vi "log queue utility.vi"(10 "array":string[](array[string]), 11 "queue with message cluster":refnum<queue>) -> (3 "appended array":string[](array[string]))   [LabVIEW 2025]
uses:
  support/Message Queue/Message Cluster_TICO behavior.ctl
panel:
  # "feed output array back into input array wiring node to create feedback element"
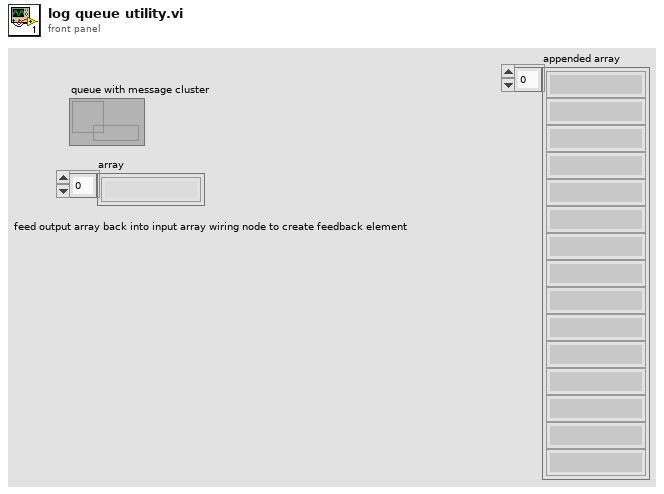
[diagram p1: front panel]
types:
  T1 = typedef "Message Cluster_TICO behavior.ctl" = cluster{"Message":string, "Message Data":variant}
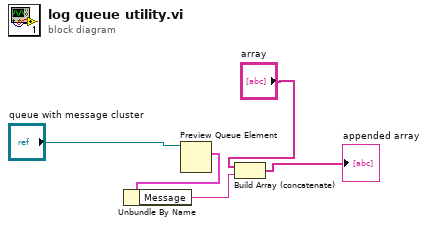
[diagram p0: block diagram]
diagram:
  n1 = Preview Queue Element(queue="queue with message cluster") -> (element=w3:T1)  [unwired: 2 in, 3 out]
  n2 = Unbundle By Name(w3) -> ("Message"=w2:string)
  n3 = Build Array (concatenate)("array", w2) -> (→"appended array":string[])
